vi "Write_Frame.vi"(5 "fdf":bool, 6 "brs":bool, 7 "ide":bool, 8 "error in (no error)":errorcluster, 9 "data":u8[](array[numeric]), 10 "id":u32 format="%.0x", 11 "channel in":refnum<class "CANsub_Channel.lvclass">) -> (0 "error out":errorcluster, 3 "channel out":refnum<class "CANsub_Channel.lvclass">)   [LabVIEW 2021, in "CANsub_API.lvlib" / "CANsub_Channel.lvclass"]
doc: "Sends one CAN or CAN FD frame: id, data (0–8 bytes classic, up to 64 FD), ide (29-bit ID), fdf (FD frame), brs (bit rate switch). One TCP Write per call. Must be overridden. Loop-safe: no allocation, bounded time."
uses:
  CANsub_Channel.lvclass
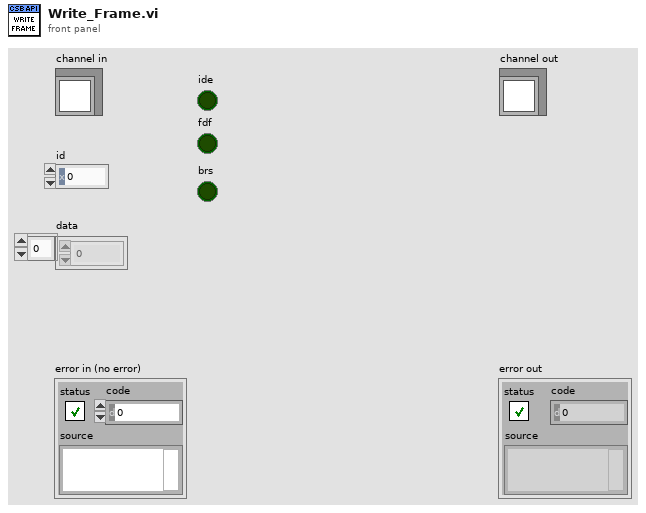
[diagram p1: front panel]
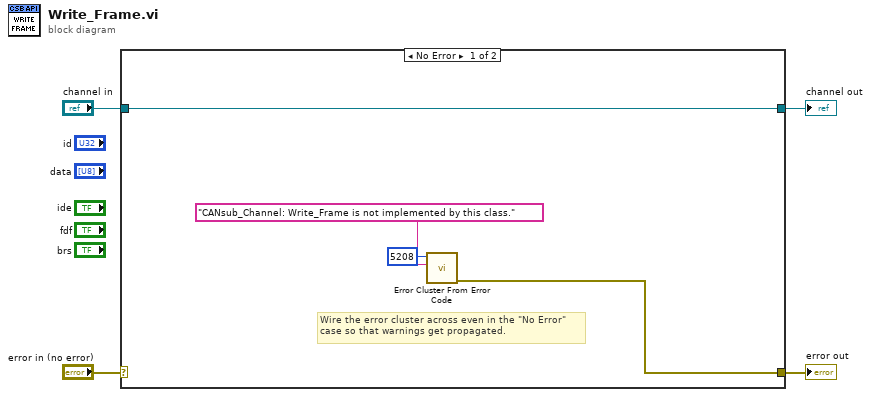
[diagram p0: block diagram]
diagram:
  n1 = case shown="No Error" "error in (no error)" {
    selector: "error in (no error)" -> [_ w10]
    tunnel: [w5 w10] -> w3
    tunnel: [w8 w9] -> w1
    tunnel: "channel in" -> [w8 w9]
    frame No Error {
      # "Wire the error cluster across even in the \"No Error\"\ncase so that warnings get propagated."
      n2 = call <vilib>:"Error Cluster From Error Code.vi"("error message (\"\")"="CANsub_Channel: Write_Frame is not implemented by this class." ("error message (\"\")"), "error code (0)"=5208) -> ("error out"=w5:errorcluster)  [unwired: 7 in]
    }
    frame Error {
    }
  }
  "error out" <- w3
  "channel out" <- w1
